vi "Open Template.vi"(8 "error in":errorcluster, 10 "Template":path, 11 "ILabVIEWFile in":refnum<class "LabVIEW File.lvclass">) -> (0 "error out":errorcluster, 3 "ILabVIEWFile out":refnum<class "LabVIEW File.lvclass">)   [LabVIEW 2026, in "LabVIEW File.lvclass"]
doc: "Open template (specified by file) and store reference in the class private data."
uses:
  LabVIEW File.lvclass
  LabVIEW File.lvclass/LabVIEW File.ctl
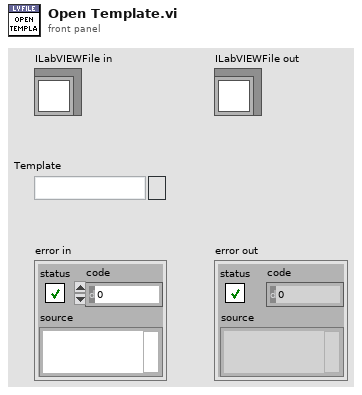
[diagram p1: front panel]
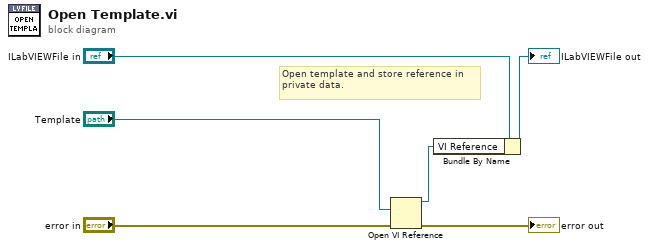
[diagram p0: block diagram]
diagram:
  # "Open template and store reference in private data."
  n1 = Open VI Reference(vi path="Template", error in (no error)="error in") -> (vi reference=w5:refnum<vi>, error out=→"error out":errorcluster)  [unwired: 4 in]
  n2 = Bundle By Name(cluster="ILabVIEWFile in", "VI Reference"=w5) -> (→"ILabVIEWFile out":refnum<class "LabVIEW File.lvclass">)
